vi "RemoteVI Client Panel.vi"(0 "geo":T3, 5 "hWnd":u64, 7 "popups":T2, 9 "popup since":u32) -> (4 "panel":T1, 6 "popup since out":u32)   [LabVIEW 2020, in "RemoteVI.lvlib"]
doc: "What servicing a client needs to know about the panel: panel = hWnd, popup (popups.windows not empty - a popup is open) and the cached geometry; popup since out = the tick count at which this client first saw the current popups open - kept while a popup stays open, now when one has just opened, 0 when none is open."
uses:
  RemoteVI.lvlib
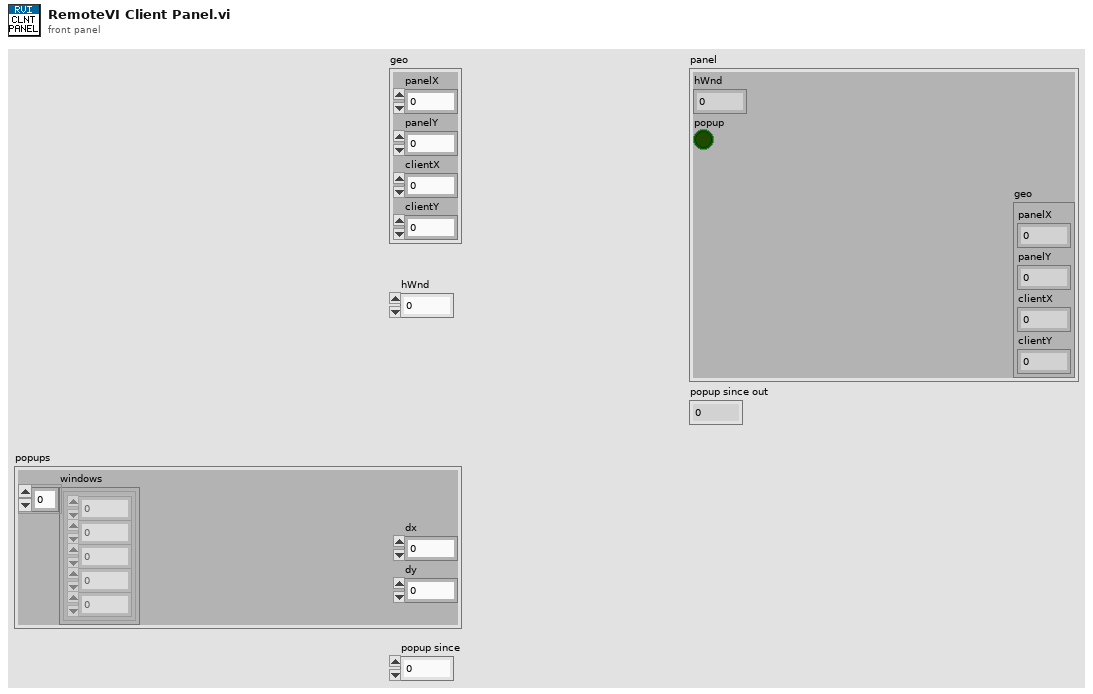
[diagram p1: front panel]
types:
  T1 = cluster{"hWnd":u64, "popup":bool, "geo":cluster{"panelX":i32, "panelY":i32, "clientX":i32, "clientY":i32}}
  T2 = cluster{"windows":cluster{"hwnd":u64, "x":i32, "y":i32, "w":i32, "h":i32}[], "dx":i32, "dy":i32}
  T3 = cluster{"panelX":i32, "panelY":i32, "clientX":i32, "clientY":i32}
  T4 = cluster{"hwnd":u64, "x":i32, "y":i32, "w":i32, "h":i32}[]
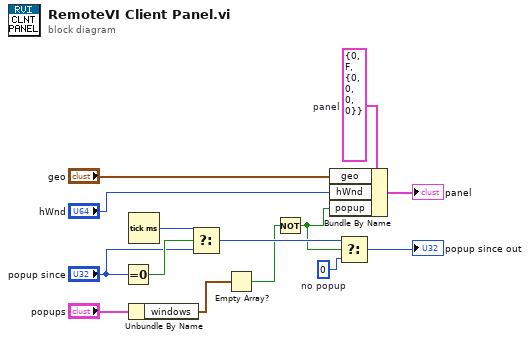
[diagram p0: block diagram]
diagram:
  w13 = u32 0  # no popup
  w8 = T1 {"hWnd"=0, "popup"=FALSE, "geo"={"panelX"=0, "panelY"=0, "clientX"=0, "clientY"=0}}  # panel
  n1 = Equal To 0?(x="popup since") -> (x = 0?=w11:bool)
  n2 = Tick Count (ms)() -> (millisecond timer value=w10:u32)
  n3 = Unbundle By Name("popups") -> ("windows"=w5:T4)
  n4 = Select(t=w10, s=w11, f="popup since") -> (s? t:f=w12:u32)
  n5 = Empty Array?(array=w5) -> (empty?=w6:bool)
  n6 = Not(x=w6) -> (.not. x?=w7:bool)
  n7 = Bundle By Name(cluster=w8, "geo"="geo", "hWnd"="hWnd", "popup"=w7) -> (→"panel":T1)
  n8 = Select(t=w12, s=w7, f=w13) -> (s? t:f=→"popup since out":u32)
